vi "init Call Box Device.vi"(8 "error in (no error)":errorcluster, 9 "Device - Protocol":T1, 10 "VISA Address":refnum<visa-resource-name>, 11 "Anritsu Call Box_Implement in":refnum<class "Anritsu Call Box_Implement.lvclass">) -> (0 "error out":errorcluster, 2 "Connected":bool, 3 "Anritsu Call Box_Implement out":refnum<class "Anritsu Call Box_Implement.lvclass">)   [LabVIEW 2023, in "ANRITSU Call Box.lvlib" / "Anritsu Call Box_Implement.lvclass"]
uses:
  Anritsu Call Box_Implement.lvclass
  Type Definition/Call Device - Protocol Type Selector.ctl
  NR/NR.lvclass
  NR/NR.lvclass/NR.ctl
  Anritsu Call Box_Implement.lvclass/Anritsu Call Box_Implement.ctl
  LTE/LTE.lvclass
  LTE/LTE.lvclass/LTE.ctl
  ANRITSU Call Box.lvlib
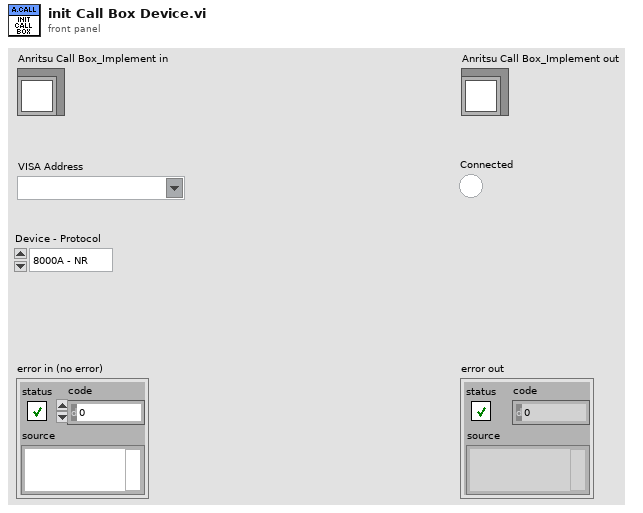
[diagram p1: front panel]
types:
  T1 = typedef "ANRITSU Call Box.lvlib/Call Device - Protocol Type Selector.ctl" = enum16{"8000A - NR", "8000A - LTE", "882xC - LTE"}
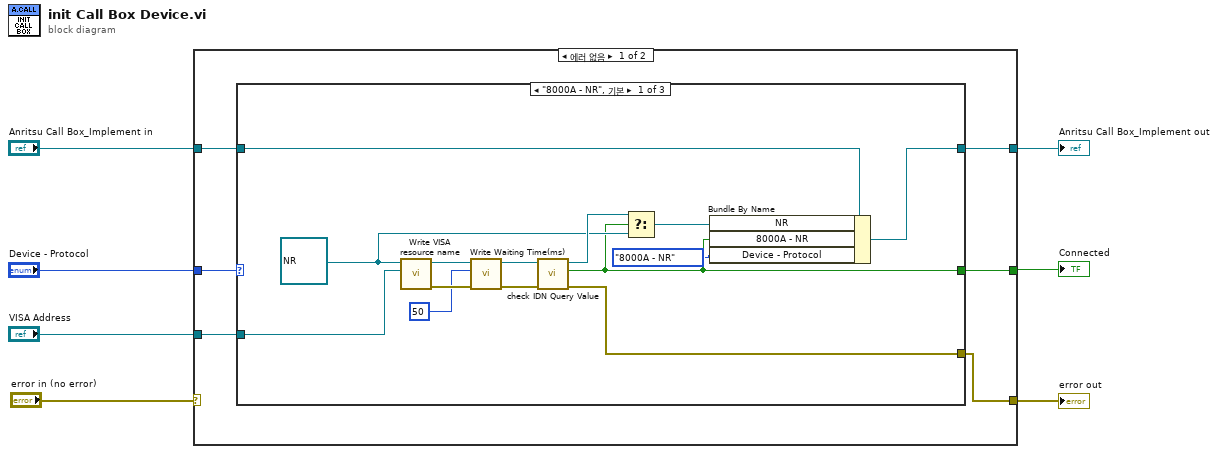
[diagram p0: block diagram]
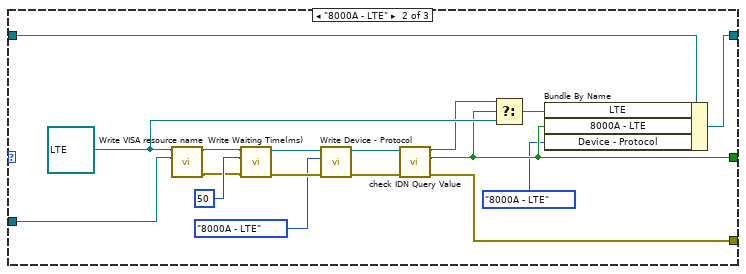
[diagram p2: hidden frame]
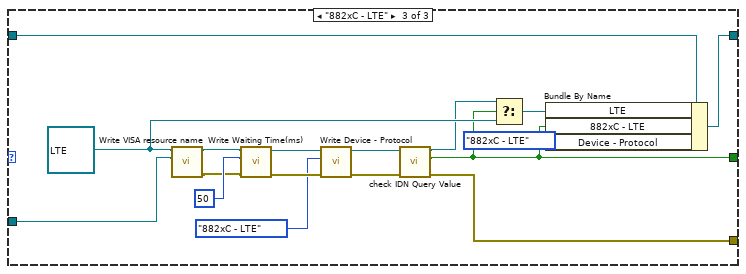
[diagram p3: hidden frame]
diagram:
  n1 = case shown="에러 없음" "error in (no error)" {
    selector: "error in (no error)" -> [_ w62]
    tunnel: "Anritsu Call Box_Implement in" -> [w11 w63]
    tunnel: [w10 w63] -> w5
    tunnel: "Device - Protocol" -> [w13 _]
    tunnel: "VISA Address" -> [w12 _]
    tunnel: [w9 _] -> w2
    tunnel: [w8 w62] -> w1
    frame No Error {
      n2 = case shown="\"8000A - NR\", 기본" w13 {
        tunnel: w12 -> [w27 w40 w57]
        tunnel: w11 -> [w19 w44 w61]
        tunnel: [w17 w42 w59] -> w10
        tunnel: [w16 w31 w48] -> w8
        tunnel: [w15 w29 w46] -> w9
        frame "8000A - NR", Default {
          w20 = refnum<class "NR.lvclass"> refnum ("ANRITSU Call Box.lvlib:NR.lvclass")
          n3 = call "Write VISA resource name.vi"("VISA resource name"=w27, "NR in"=w20) -> ("error out"=w25:errorcluster, "NR out"=w26:refnum<class "NR.lvclass">)  [unwired: 8 in]
          n4 = call "Write Waiting Time(ms).vi"("error in (no error)"=w25, "Waiting Time(ms)"=u32 50, "NR in"=w26) -> ("error out"=w22:errorcluster, "NR out"=w23:refnum<class "NR.lvclass">)  [unwired: 7 in]
          n5 = call "check IDN Query Value.vi"("error in (no error)"=w22, "NR in"=w23) -> ("error out"=w16:errorcluster, "Connected"=w15:bool, "NR out"=w21:refnum<class "NR.lvclass">)  [unwired: 7 in]
          n6 = Select(t=w21, s=w15, f=w20) -> (s? t:f=w18:refnum<class "NR.lvclass">)
          n7 = Bundle By Name(cluster=w19, "NR"=w18, "8000A - NR"=w15, "Device - Protocol"=Call_Device_-_Protocol_Type_Selector."8000A - NR") -> (w17:refnum<class "Anritsu Call Box_Implement.lvclass">)
        }
        frame "8000A - LTE" {
          w41 = refnum<class "LTE.lvclass"> refnum ("ANRITSU Call Box.lvlib:LTE.lvclass")
          n8 = call "Write VISA resource name.vi"("VISA resource name"=w40, "LTE in"=w41) -> ("error out"=w37:errorcluster, "LTE out"=w39:refnum<class "LTE.lvclass">)  [unwired: 8 in]
          n9 = call "Write Waiting Time(ms).vi"("error in (no error)"=w37, "Waiting Time(ms)"=u32 50, "LTE in"=w39) -> ("error out"=w35:errorcluster, "LTE out"=w36:refnum<class "LTE.lvclass">)  [unwired: 7 in]
          n10 = call "Write Device - Protocol.vi"("error in (no error)"=w35, "Device - Protocol"=Call_Device_-_Protocol_Type_Selector."8000A - LTE", "LTE in"=w36) -> ("error out"=w32:errorcluster, "LTE out"=w33:refnum<class "LTE.lvclass">)  [unwired: 7 in]
          n11 = call "check IDN Query Value.vi"("error in (no error)"=w32, "LTE in"=w33) -> ("error out"=w31:errorcluster, "Connected"=w29:bool, "LTE out"=w30:refnum<class "LTE.lvclass">)  [unwired: 7 in]
          n12 = Select(t=w30, s=w29, f=w41) -> (s? t:f=w43:refnum<class "LTE.lvclass">)
          n13 = Bundle By Name(cluster=w44, "LTE"=w43, "8000A - LTE"=w29, "Device - Protocol"=Call_Device_-_Protocol_Type_Selector."8000A - LTE") -> (w42:refnum<class "Anritsu Call Box_Implement.lvclass">)
        }
        frame "882xC - LTE" {
          w58 = refnum<class "LTE.lvclass"> refnum ("ANRITSU Call Box.lvlib:LTE.lvclass")
          n14 = call "Write VISA resource name.vi"("VISA resource name"=w57, "LTE in"=w58) -> ("error out"=w54:errorcluster, "LTE out"=w56:refnum<class "LTE.lvclass">)  [unwired: 8 in]
          n15 = call "Write Waiting Time(ms).vi"("error in (no error)"=w54, "Waiting Time(ms)"=u32 50, "LTE in"=w56) -> ("error out"=w52:errorcluster, "LTE out"=w53:refnum<class "LTE.lvclass">)  [unwired: 7 in]
          n16 = call "Write Device - Protocol.vi"("error in (no error)"=w52, "Device - Protocol"=Call_Device_-_Protocol_Type_Selector."882xC - LTE", "LTE in"=w53) -> ("error out"=w49:errorcluster, "LTE out"=w50:refnum<class "LTE.lvclass">)  [unwired: 7 in]
          n17 = call "check IDN Query Value.vi"("error in (no error)"=w49, "LTE in"=w50) -> ("error out"=w48:errorcluster, "Connected"=w46:bool, "LTE out"=w47:refnum<class "LTE.lvclass">)  [unwired: 7 in]
          n18 = Select(t=w47, s=w46, f=w58) -> (s? t:f=w60:refnum<class "LTE.lvclass">)
          n19 = Bundle By Name(cluster=w61, "LTE"=w60, "882xC - LTE"=w46, "Device - Protocol"=Call_Device_-_Protocol_Type_Selector."882xC - LTE") -> (w59:refnum<class "Anritsu Call Box_Implement.lvclass">)
        }
      }
    }
    frame Error {
    }
  }
  "error out" <- w1
  "Anritsu Call Box_Implement out" <- w5
  "Connected" <- w2
